vi "EJERCICIO _2_WHILE_CASE.vi"() -> ()   [LabVIEW 2026]
panel:
  in  "PARAR":bool
  out "ALARMA":bool
  in  "TEMPERATURA":dbl
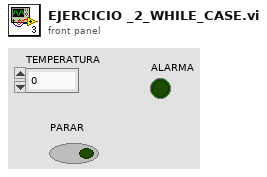
[diagram p1: front panel]
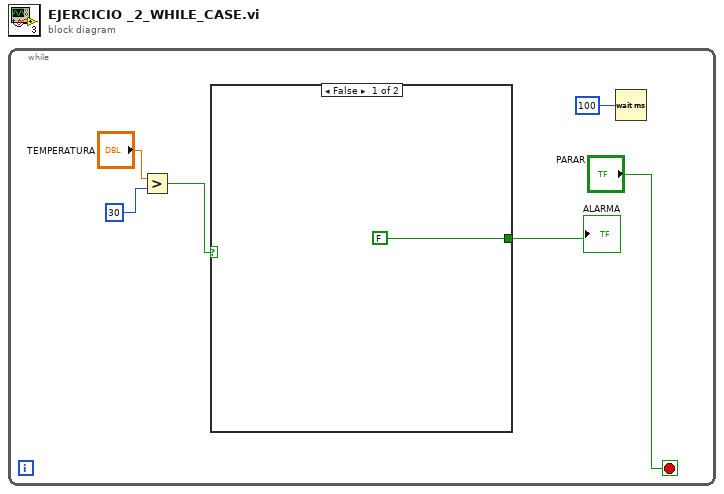
[diagram p0: block diagram]
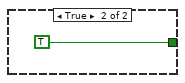
[diagram p2: hidden frame]
diagram:
  n1 = while {
    stop <- "PARAR" stop-if-true
    n2 = Greater?(x="TEMPERATURA", y=30) -> (0:w4:bool)
    n3 = case shown="False" w4 {
      tunnel: [FALSE TRUE] -> w3
      frame False {
      }
      frame True {
      }
    }
    "ALARMA" <- w3
    n4 = Wait (ms)(milliseconds to wait=100) -> ()  [unwired: 1 out]
  }
